vi "RemoteVI Cross Origin.vi"(0 "origin exists?":bool, 5 "origin":string, 7 "host":string) -> (4 "cross origin?":bool)   [LabVIEW 2020, in "RemoteVI.lvlib"]
doc: "TRUE when a request carries an Origin header that names another host than its Host header: the part of origin after \"://\" is compared with host. A request without an Origin header (origin exists? FALSE) is never cross-origin. Used by RemoteVI Handle Connection.vi to answer a cross-origin WebSocket upgrade with 403 (docs\\security.md). Pure."
uses:
  RemoteVI.lvlib
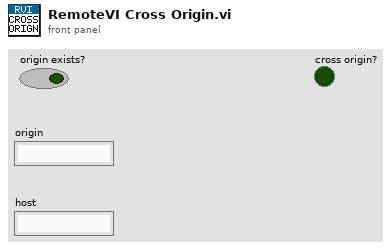
[diagram p1: front panel]
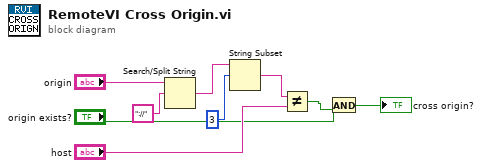
[diagram p0: block diagram]
diagram:
  n1 = Search/Split String(string="origin", search string/char (-)="://") -> (match + rest of string=w5:string)  [unwired: 1 in, 2 out]
  n2 = String Subset(string=w5, offset (0)=3) -> (substring=w7:string)  [unwired: 1 in]
  n3 = Not Equal?(x=w7, y="host") -> (x != y?=w8:bool)
  n4 = And(x="origin exists?", y=w8) -> (x .and. y?=→"cross origin?":bool)
